vi "Start Test.vi"(8 "error in (no error)":errorcluster, 10 "Tests":string[](array[string]), 11 "Text Report In":refnum<class "Text Report.lvclass">) -> (0 "error out":errorcluster, 3 "Text Report Out":refnum<class "Text Report.lvclass">)   [LabVIEW 2020, in "Text Report.lvclass"]
uses:
  Text Report.lvclass
  C:/git/astemes-lunit/source/Framework/Report Plugin/Report Plugin.lvclass
  Text Report.lvclass/Text Report.ctl
  Framework/Report Plugin/Report Plugin.lvclass
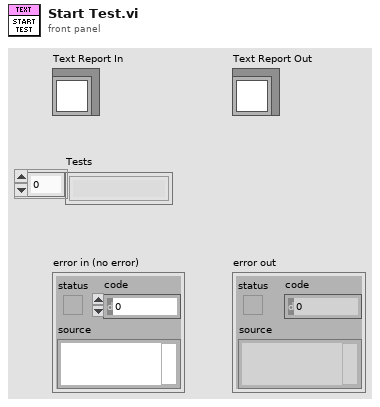
[diagram p1: front panel]
types:
  T1 = enum16{"open", "replace", "create", "open or create", "replace or create", "replace or create with confirmation"}
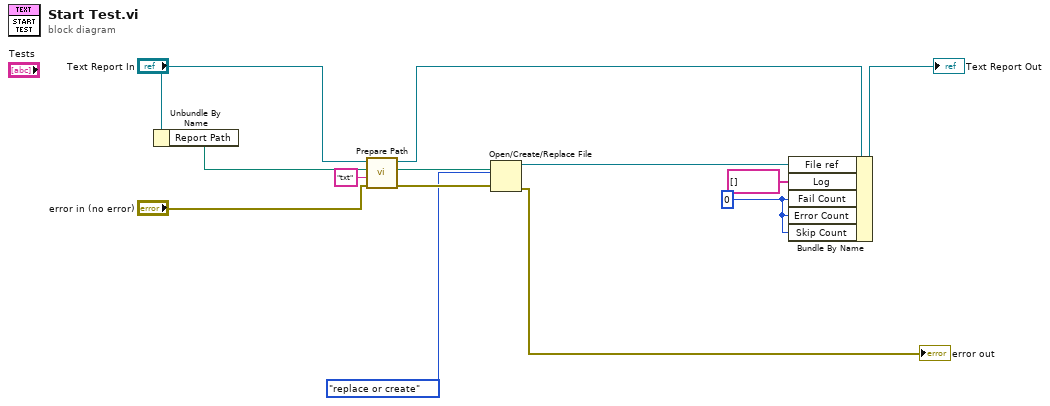
[diagram p0: block diagram]
diagram:
  w11 = 0 ("Fail Count")
  n1 = Unbundle By Name("Text Report In") -> ("Report Path"=w8:path)
  n2 = call "Prepare Path.vi"("error in (no error)"="error in (no error)", "Extenssion"="txt", "File Path in"=w8, "Plugin In"="Text Report In") -> ("error out"=w4:errorcluster, "Modified Path"=w5:path, "Plugin Out"=w9:refnum<class "Text Report.lvclass">)  [unwired: 5 in]
  n3 = Open/Create/Replace File(file path (use dialog)=w5, error in=w4, operation (0:open)=T1."replace or create") -> (refnum out=w2:refnum<file>, error out=→"error out":errorcluster)  [unwired: 3 in, 1 out]
  n4 = Bundle By Name(cluster=w9, "File ref"=w2, "Log"=string[] [], "Fail Count"=w11, "Error Count"=w11, "Skip Count"=w11) -> (→"Text Report Out":refnum<class "Text Report.lvclass">)
